vi "Initialize DeepU Panel.vi"() -> (0 "error out":errorcluster, 2 "DeepU Results queue out":refnum<queue>, 3 "Event Registration Refnum":refnum<event-registration>)   [LabVIEW 2019, in "Test Stands.lvlib" / "DeepU Test Stand.lvclass"]
uses:
  DeepU Test Stand.lvclass
  Results/DeepU Results/DeepU Results.lvclass
  C:/Users/wg/Documents/LV_Projects/test-stand/App/Generic Test Stand/Generic Test Stand.lvclass
  Generic Test Stand/Generic Test Stand.lvclass/Generic Test Stand.ctl
  DeepU Test Stand.lvclass/DeepU Test Stand.ctl
  Generic Test Stand/Generic Test Stand.lvclass
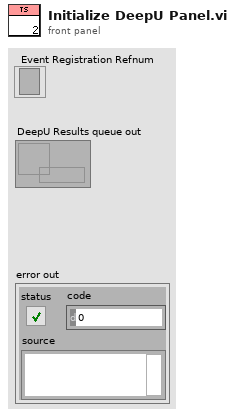
[diagram p1: front panel]
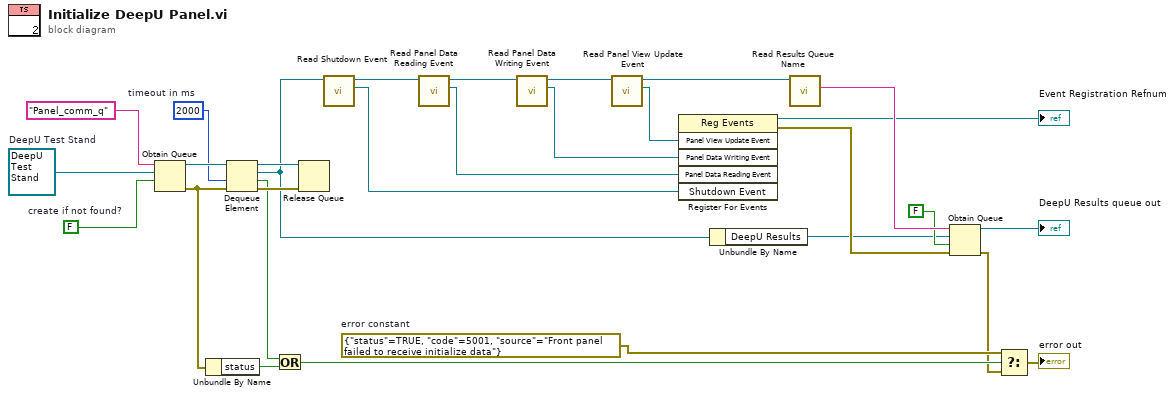
[diagram p0: block diagram]
diagram:
  w11 = refnum<class "DeepU Test Stand.lvclass"> refnum  # DeepU Test Stand
  w17 = errorcluster {"status"=TRUE, "code"=5001, "source"="Front panel failed to receive initialize data"}  # error constant
  w26 = 2000  # timeout in ms
  w28 = FALSE  # create if not found?
  n1 = Obtain Queue(name (unnamed)="Panel_comm_q", element data type=w11, create if not found? (T)=w28) -> (queue out=w27:refnum<queue>, error out=w21:errorcluster)  [unwired: 2 in, 1 out]
  n2 = Unbundle By Name(w21) -> ("status"=w20:bool)
  n3 = Dequeue Element(queue=w27, timeout in ms (-1)=w26, error in (no error)=w21) -> (queue out=w25:refnum<queue>, element=w10:refnum<class "DeepU Test Stand.lvclass">, timed out?=w19:bool, error out=w24:errorcluster)
  n4 = Or(x=w19, y=w20) -> (x .or. y?=w18:bool)
  n5 = Release Queue(queue=w25, error in (no error)=w24) -> ()  [unwired: 1 in, 3 out]
  n6 = call "Read Shutdown Event.vi"("Generic Test Stand in"=w10) -> ("Shutdown Event"=w7:refnum<user-event>, "Generic Test Stand out"=w23:refnum<class "DeepU Test Stand.lvclass">)  [unwired: 8 in, 1 out]
  n7 = call "Read Panel Data Reading Event.vi"("Generic Test Stand in"=w23) -> ("Panel Data Reading Event"=w6:refnum<user-event>, "Generic Test Stand out"=w22:refnum<class "DeepU Test Stand.lvclass">)  [unwired: 8 in, 1 out]
  n8 = call "Read Panel Data Writing Event.vi"("Generic Test Stand in"=w22) -> ("Panel Data Writing Event"=w5:refnum<user-event>, "Generic Test Stand out"=w4:refnum<class "DeepU Test Stand.lvclass">)  [unwired: 8 in, 1 out]
  n9 = call "Read Panel View Update Event.vi"("Generic Test Stand in"=w4) -> ("Panel View Update Event"=w2:refnum<user-event>, "Generic Test Stand out"=w3:refnum<class "DeepU Test Stand.lvclass">)  [unwired: 8 in, 1 out]
  n10 = register-events(w2, w5, w6, w7) -> (reference out=→"Event Registration Refnum":refnum<event-registration>, error out=w12:errorcluster)  [unwired: 2 in]
  n11 = Unbundle By Name(w10) -> ("DeepU Results"=w9:refnum<class "DeepU Results.lvclass">)
  n12 = call "Read Results Queue Name.vi"("Generic Test Stand in"=w3) -> ("Results Queue Name"=w15:string)  [unwired: 8 in, 2 out]
  n13 = Obtain Queue(name (unnamed)=w15, element data type=w9, create if not found? (T)=FALSE, error in (no error)=w12) -> (queue out=→"DeepU Results queue out":refnum<queue>, error out=w13:errorcluster)  [unwired: 1 in, 1 out]
  n14 = Select(t=w17, s=w18, f=w13) -> (s? t:f=→"error out":errorcluster)
